vi "Acquire Data.vi"(7 "user event":T2, 8 "error in (no error)":errorcluster, 9 "UI Refs":T1, 10 "Waveforms":waveform(dbl)[](array[waveform]), 11 "H1Velocity":refnum<class "H1 Velocity.lvclass">) -> (0 "error out":errorcluster, 3 "H1Velocity out":refnum<class "H1 Velocity.lvclass">)   [LabVIEW 2025, in "H1 Plotter.lvlib" / "H1 Velocity.lvclass"]
uses:
  H1 Velocity.lvclass
  Users/Public/Documents/Sandia National Labs/TSS Plugin/CEF.lvlibp/Node/UserEventRef.ctl
  H1 Velocity.lvclass/H1 Velocity.ctl
  Users/Public/Documents/Sandia National Labs/TSS Plugin/Tests/XY Plotter.lvlibp/XY Plotter configuration/Read XY Plotter.vi
  Users/Public/Documents/Sandia National Labs/TSS Plugin/CEF.lvlibp/serializable configuration/CEF_serializable configuration.lvclass
  Users/Public/Documents/Sandia National Labs/TSS Plugin/Tests/XY Plotter.lvlibp/XY Plotter configuration/XY Plotter configuration.lvclass
  <vilib>/Analysis/baseanly.llb/Mean (DBL).vi
  <vilib>/Analysis/NI_AALBase.lvlib
  Users/Public/Documents/Sandia National Labs/TSS Plugin/Tests/XY Plotter.lvlibp/XY  Plotter/XY Plotter.lvclass
  Users/Public/Documents/Sandia National Labs/TSS Plugin/CEF.lvlibp/Node/CEF_Node.lvclass
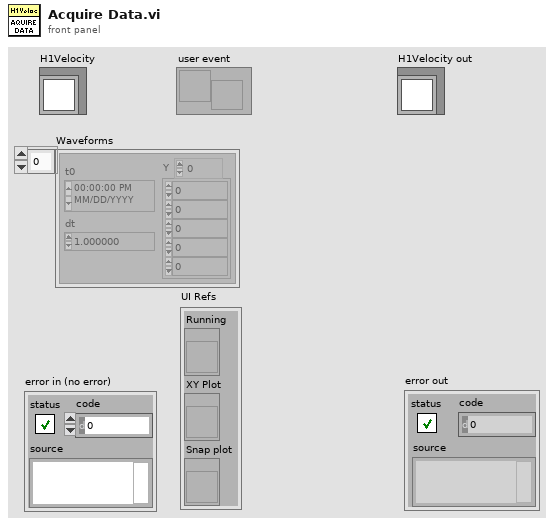
[diagram p1: front panel]
types:
  T1 = cluster{"Running":refnum<vi>, "XY Plot":refnum<vi>, "Snap plot":refnum<vi>}
  T2 = typedef "CEF.lvlibp/CEF_Node.lvclass/UserEventRef.ctl" = refnum<user-event>
  T3 = typedef "XY Plotter.lvlibp/XY Plotter configuration.lvclass/XY Plotter.ctl" = cluster{"Data Rate":i32, "Y-Scales":cluster{"Label":string, "Max":dbl, "Min":dbl, "Unit":enum16{"---", "V", "mA", "sec", "dB", "deg", "in/s", "in", "lbf", "Hz", "psi", "gpm"}, "Visible":bool}[], "Note":string, "History Length":i32, "DataLog Path":path, "Plot type":bool, "X-Scales":cluster{"Label":string, "Max":dbl, "Min":dbl, "Unit":enum16{"---", "V", "mA", "sec", "dB", "deg", "in/s", "in", "lbf", "Hz", "psi", "gpm"}, "Visible":bool}[], "Plot List":cluster{"Plot Name":string, "X Scale Index":u32, "Y Scale Index":u32, "Visible":bool}[]}
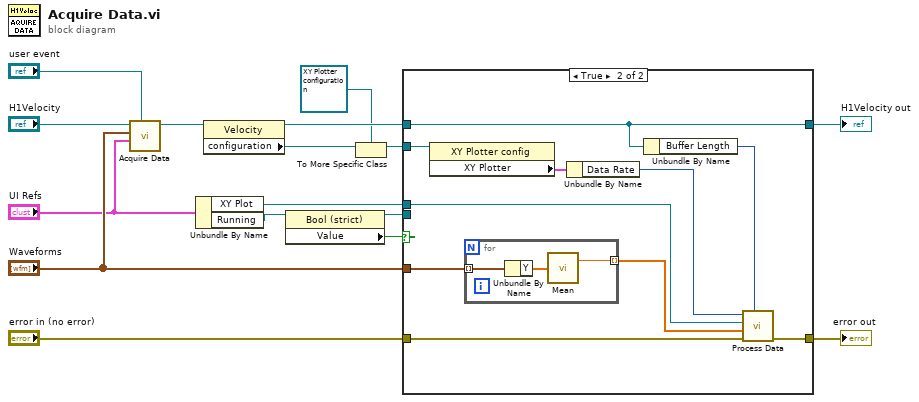
[diagram p0: block diagram]
diagram:
  n1 = call-parent "Acquire Data.vi"("user event"="user event", "UI Refs"="UI Refs", "Waveforms"="Waveforms", "XY Plotter"="H1Velocity") -> ("XY Plotter out"=w4:refnum<class "H1 Velocity.lvclass">)  [unwired: 6 in, 1 out]
  n2 = Unbundle By Name("UI Refs") -> ("XY Plot"=w8:refnum<vi>, "Running"=w9:refnum<vi>)
  n3 = property class="Velocity"(reference=w4) -> (reference out=w12:refnum<class "H1 Velocity.lvclass">, "configuration"=w7:refnum<class "CEF_serializable configuration.lvclass">)  [unwired: 1 in, 1 out]
  n4 = property class="Bool (strict)"(reference=w9) -> (reference out=w15:refnum<vi>, "Value"=w16:bool)  [unwired: 1 in, 1 out]
  n5 = To More Specific Class(target class=refnum<class "XY Plotter configuration.lvclass"> refnum ("XY Plotter.lvlibp:XY Plotter config"), reference=w7) -> (specific class reference=w5:refnum<class "XY Plotter configuration.lvclass">)  [unwired: 1 in, 1 out]
  n6 = case shown="True" w16 {
    tunnel: [w18 w28] -> w10
    tunnel: w15 -> [_ _]
    tunnel: w12 -> [w18 w28]
    tunnel: "error in (no error)" -> [w17 w25]
    tunnel: [w17 w22] -> w14
    tunnel: "Waveforms" -> [_ w27]
    tunnel: w8 -> [_ w26]
    tunnel: w5 -> [_ w23]
    frame False {
    }
    frame True {
      n7 = property class="XY Plotter config"(reference=w23) -> ("XY Plotter"=w24:T3)  [unwired: 1 in, 2 out]
      n8 = for {
        tunnel: w27 -> [w31] mode=indexing
        tunnel: [w29] -> w20 mode=indexing
        n9 = Unbundle By Name(w31) -> ("Y"=w30:dbl[])
        n10 = call-poly <vilib>:"Mean.vi"("X"=w30) -> ("mean"=w29:dbl)  [unwired: 1 out]
      }
      n11 = Unbundle By Name(w24) -> ("Data Rate"=w19:i32)
      n12 = Unbundle By Name(w28) -> ("Buffer Length"=w21:i32)
      n13 = call "Process Data.vi"("Buffer Length"=w21, "error in (no error)"=w25, "Data"=w20, "XY Plot"=w26, "Data Rate"=w19) -> ("error out"=w22:errorcluster)  [unwired: 6 in]
    }
  }
  "error out" <- w14
  "H1Velocity out" <- w10
